vi "Parallel Process Markov Chains.vi"(6 "Suggestion Limit":u16=4, 7 "Queue in":refnum<queue>, 8 "error in (no error)":errorcluster, 9 "Parallel Instances (8)":i32=8, 10 "Progress ref in":refnum<vi>, 11 "Pattern Frequencies":map{string[], i32}(c390)) -> (0 "error out":errorcluster, 3 "Map":T1(c390))   [LabVIEW 2020]
uses:
  <vilib>/Utility/miscctls.llb/LVMapReplaceAction.ctl
  Indexer Action.ctl
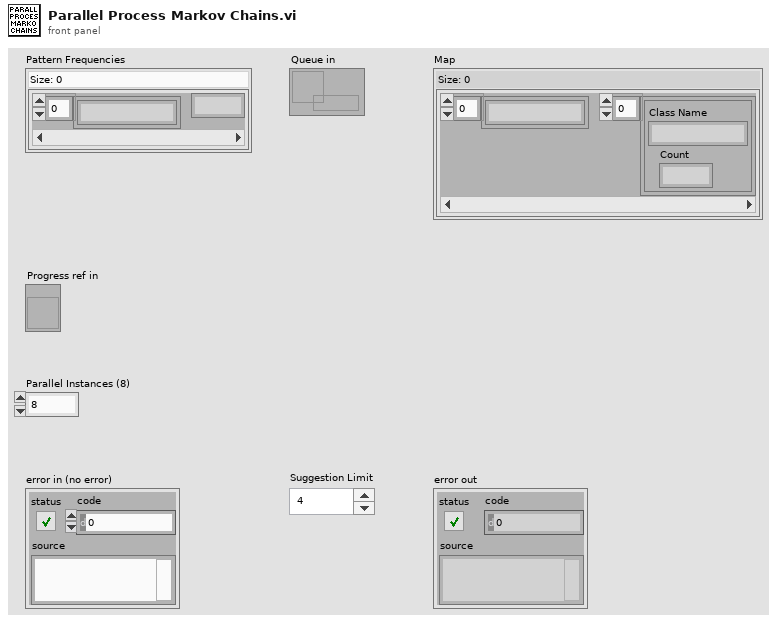
[diagram p1: front panel]
types:
  T1 = map{string[], cluster{"Class Name":string, "Count":i32}[]}
  T2 = map{string[], cluster{"Count":i32, "Class Name":string}[]}
  T3 = typedef "LVMapReplaceAction.ctl" = enum32{"Modify Entry only if found", "Add or Modify Entry", "Delete Entry"}
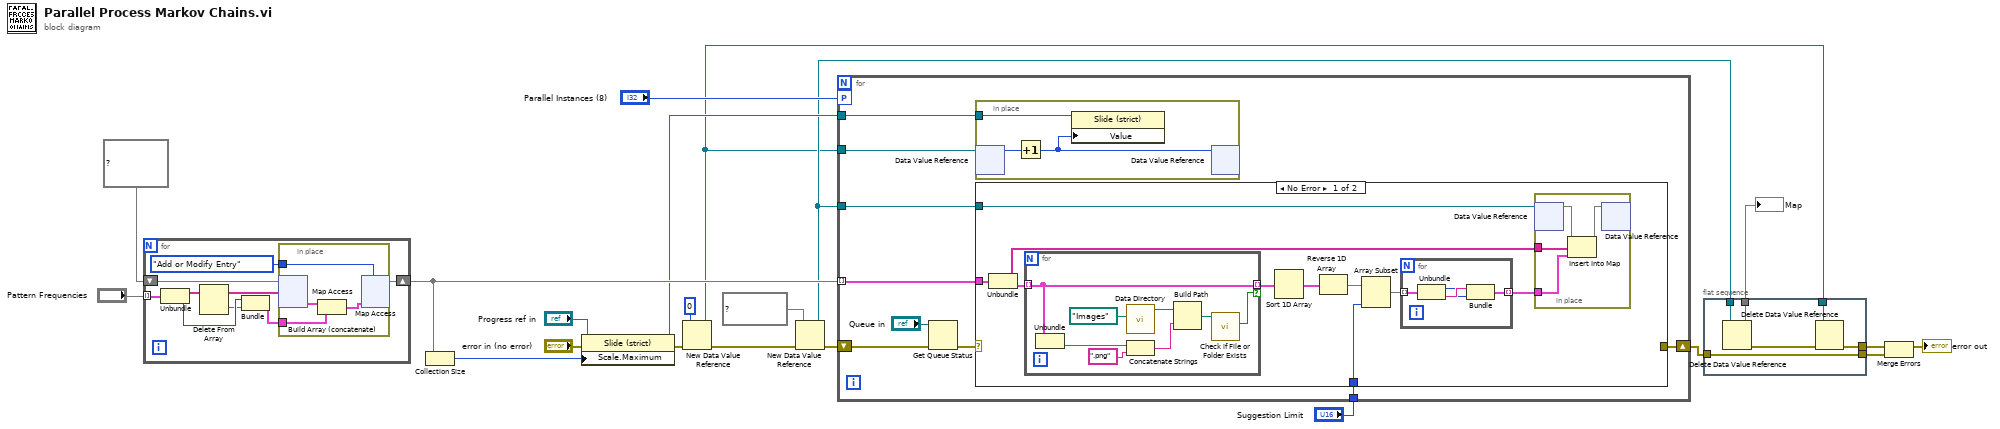
[diagram p0: block diagram]
diagram:
  n1 = for {
    tunnel: "Pattern Frequencies" -> [w30] mode=indexing
    shift-right: [w25] -> w20
    shift-left: T2 {} ("Map") -> [w26]
    n2 = Unbundle(w30) -> (w29:string[], w24:i32)
    n3 = Delete From Array(array=w29) -> (deleted portion=w23:string, array with subset deleted=w28:string[])  [unwired: 2 in]
    n4 = Bundle(w24, "Class Name"=w23) -> (w27:cluster{i32, "Class Name":string})  [unwired: 1 in]
    n5 = in-place {
      in-place-border: w27 -> [w33]
      in-place-border: LVMapReplaceAction."Add or Modify Entry" ("action") -> [w31]
      n6 = in-place-map #1(w26, w28) -> (w34:cluster{"Count":i32, "Class Name":string}[])  [unwired: 1 in, 1 out]
      n7 = Build Array (concatenate)(w34, w33) -> (w32:cluster{"Count":i32, "Class Name":string}[])
      n8 = in-place-map #1(w32, w31) -> (w25:T2)  [unwired: 2 out]
    }
  }
  n9 = Collection Size(1:w20) -> (0:w14:i32)
  n10 = property on="Property Node" class="Slide (strict)"(reference="Progress ref in", error in="error in (no error)", "Scale.Maximum"=w14) -> (reference out=w12:refnum<vi>, error out=w15:errorcluster)
  n11 = New Data Value Reference(data value=u64 0, error in=w15) -> (data value reference=w1:refnum<data-value>, error out=w9:errorcluster)
  n12 = New Data Value Reference(data value=T1 {} ("Map"), error in=w9) -> (data value reference=w2:refnum<data-value>, error out=w10:errorcluster)
  n13 = for {
    tunnel: w20 -> [w43] mode=indexing
    tunnel: "Suggestion Limit" -> [w42]
    shift-right: [w39] -> w3
    shift-left: w10 -> [w40]
    workers-P: "Parallel Instances (8)" -> [_]
    tunnel: w1 -> [w38]
    tunnel: w12 -> [w36]
    tunnel: w2 -> [w35]
    n14 = Get Queue Status(queue="Queue in", error in (no error)=w40) -> (error out=w41:errorcluster)  [unwired: 1 in, 7 out]
    n15 = in-place {
      in-place-border: w36 -> [w45]
      n16 = in-place-dvr #2(w38) -> (w46:u64)  [unwired: 1 out]
      n17 = Increment(x=w46) -> (x+1=w44:u64)
      n18 = property class="Slide (strict)"(reference=w45, "Value"=w44) -> ()  [unwired: 1 in, 2 out]
      n19 = in-place-dvr #2(w44) -> ()  [unwired: 2 out]
    }
    n20 = case shown="No Error" w41 {
      selector: w41 -> [_ w73]
      tunnel: w43 -> [w56 _]
      tunnel: w42 -> [w50 _]
      tunnel: [_ w73] -> w39
      tunnel: w35 -> [w49 _]
      frame No Error {
        n21 = Unbundle(w56) -> (w48:string[], w52:cluster{"Count":i32, "Class Name":string}[])
        n22 = for {
          tunnel: w52 -> [w68] mode=indexing
          tunnel: [w68] -> w51 mode=indexing if=w63
          n23 = Unbundle(w68) -> ("Class Name"=w64:string)  [unwired: 1 out]
          n24 = call "Data Directory.vi"("Subdirectory"=path "Images" ("name or relative path")) -> ("Data directory"=w61:path)  [unwired: 9 in, 1 out]
          n25 = Concatenate Strings(w64, ".png" ("string")) -> (w66:string)
          n26 = Build Path(base path=w61, name or relative path=w66) -> (appended path=w67:path)
          n27 = call <vilib>:"Check if File or Folder Exists.vi"("path"=w67) -> ("file or folder exists?"=w63:bool)  [unwired: 8 in, 2 out]
        }
        n28 = Sort 1D Array(array=w51) -> (sorted array=w54:cluster{"Count":i32, "Class Name":string}[])
        n29 = Reverse 1D Array(array=w54) -> (reversed array=w53:cluster{"Count":i32, "Class Name":string}[])
        n30 = Array Subset(array=w53, length=w50) -> (w55:cluster{"Count":i32, "Class Name":string}[])  [unwired: 1 in]
        n31 = for {
          tunnel: w55 -> [w72] mode=indexing
          tunnel: [w71] -> w47 mode=indexing
          n32 = Unbundle(w72) -> ("Count"=w69:i32, "Class Name"=w70:string)
          n33 = Bundle("Class Name"=w70, "Count"=w69) -> (w71:cluster{"Class Name":string, "Count":i32})  [unwired: 1 in]
        }
        n34 = in-place {
          in-place-border: w48 -> [w58]
          in-place-border: w47 -> [w57]
          n35 = in-place-dvr #3(w49) -> (w60:T1)  [unwired: 1 out]
          n36 = Insert Into Map(map in=w60, key=w58, value=w57) -> (map out=w59:T1)  [unwired: 2 out]
          n37 = in-place-dvr #3(w59) -> ()  [unwired: 2 out]
        }
      }
      frame Error {
      }
    }
  }
  n38 = flat-sequence {
    tunnel: w1 -> [w79]
    tunnel: w2 -> [w77]
    tunnel: [w76] -> w6
    tunnel: [w75] -> w5
    tunnel: [w74] -> w4
    tunnel: w3 -> [w74]
    frame #0 {
      n39 = Delete Data Value Reference(data value reference=w77) -> (data value=w75:T1, error out=w78:errorcluster)  [unwired: 1 in]
      n40 = Delete Data Value Reference(data value reference=w79, error in=w78) -> (error out=w76:errorcluster)  [unwired: 1 out]
    }
  }
  n41 = Merge Errors(w6, w4) -> (→"error out":errorcluster)
  "Map" <- w5
